vi "TCP Server Launch Listener Process.vi"(8 "error out":errorcluster, 11 "RefNum":refnum<class "JKI TCP Server.lvclass">) -> (0 "error":errorcluster, 3 "dup RefNum":refnum<class "JKI TCP Server.lvclass">)   [LabVIEW 2020, in "JKI TCP Server.lvclass"]
uses:
  JKI TCP Server.lvclass
  _Processes/TCP Server Listener Process.vi
  JKI TCP Server.lvclass/JKI TCP Server.ctl
panel:
  # "Copyright © 2004-2008 JKI. All rights reserved.\n\nAuthor: Jim Kring [jim.kring@jameskring.com]\n\nThis library is provided \"AS IS\" ,WITHOUT WARRANTIES OR \nCONDITIONS OF ANY KIND, either express or implied.\n\nJames Kring, Inc. -- http://www.jameskring.com"
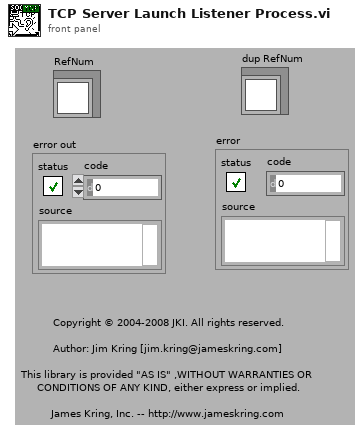
[diagram p1: front panel]
types:
  T1 = typedef "JKI TCP Server.lvclass/TCP Server Data.ctl" = cluster{"Listener Info":T2, "Connection Process VI RefNums":refnum<vi>[], "dup connection IDs (for quick search)":refnum<k5>[], "Connections":T3[], "Connection Handler VI Path":path, "Handler Is Reentrant?":bool, "TCP Handler Instance RefNums":T4[], "TCP Handler VI RefNum":T4, "No. Connections":u32, "Max Connections":u32, "server start time":u32, "Additional Data":variant}
  T2 = typedef "JKI TCP Server.lvclass/TCP Server Listener Info Cluster.ctl" = cluster{"listener ID":refnum<k5>, "net address":u32, "port":u16, "Listener Process VI Refnum":refnum<vi>}
  T3 = typedef "JKI TCP Server.lvclass/TCP Server Connection Info Cluster.ctl" = cluster{"connection ID":refnum<k5>, "Remote Address":string, "remote port":u16, "connection start time":u32}
  T4 = typedef "JKI TCP Server.lvclass/TCP Server Handler RefNum.ctl" = refnum<vi>
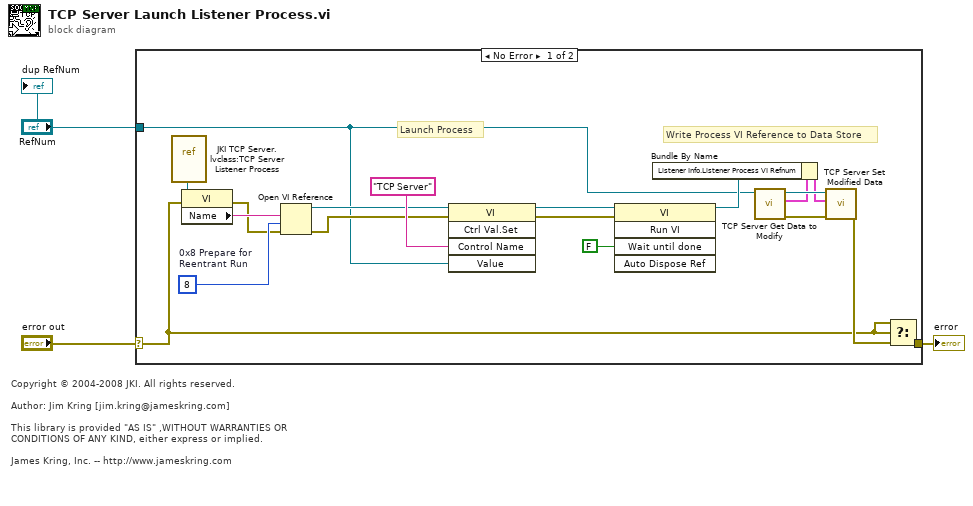
[diagram p0: block diagram]
diagram:
  # "Copyright © 2004-2008 JKI. All rights reserved.\n\nAuthor: Jim Kring [jim.kring@jameskring.com]\n\nThis library is provided \"AS IS\" ,WITHOUT WARRANTIES OR \nCONDITIONS OF ANY KIND, either express or implied.\n\nJames Kring, Inc. -- http://www.jameskring.com"
  n1 = case shown="No Error" "error out" {
    selector: "error out" -> [w5 w23]
    tunnel: [w9 w23] -> w3
    tunnel: "RefNum" -> [w8 _]
    frame No Error {
      w11 = 8  # 0x8 Prepare for Reentrant Run
      # "Write Process VI Reference to Data Store"
      # "Launch Process"
      n2 = vi-ref "JKI TCP Server.lvclass:TCP Server Listener Process.vi"() -> (w7:refnum<vi>)
      n3 = property class="VI"(reference=w7, error in=w5) -> (error out=w4:errorcluster, "Name"=w6:string)  [unwired: 1 out]
      n4 = Open VI Reference(vi path=w6, options=w11, error in (no error)=w4) -> (vi reference=w13:refnum<vi>, error out=w12:errorcluster)  [unwired: 3 in]
      n5 = invoke class="VI" method="Ctrl Val.Set"(reference=w13, error in=w12, "Control Name"="TCP Server", "Value"=w8) -> (reference out=w15:refnum<vi>, error out=w17:errorcluster)  [unwired: 1 in, 3 out]
      n6 = invoke class="VI" method="Run VI"(reference=w15, error in=w17, "Wait until done"=FALSE) -> (reference out=w21:refnum<vi>)  [unwired: 2 in, 4 out]
      n7 = call "TCP Server Get Data to Modify.vi"("RefNum"=w8) -> ("error out"=w18:errorcluster, "Data out"=w19:T1, "dup RefNum"=w22:refnum<class "JKI TCP Server.lvclass">)  [unwired: 7 in, 1 out]
      n8 = Bundle By Name(cluster=w19, "Listener Info.Listener Process VI Refnum"=w21) -> (w20:T1)
      n9 = call "TCP Server Set Modified Data.vi"("error in (no error)"=w18, "Data in"=w20, "RefNum"=w22) -> ("error out"=w10:errorcluster)  [unwired: 7 in, 1 out]
      n10 = Select(t=w5, s=w5, f=w10) -> (s? t:f=w9:errorcluster)
    }
    frame Error {
    }
  }
  "error" <- w3
  "dup RefNum" <- "RefNum"
